vi "Create Client from Template.vi"(7 "Template Library":path, 8 "error in (no error)":errorcluster, 9 "Generated Server Name":string="Generated Server", 10 "Target Project Path":path, 11 "Application ref in":refnum<vi>) -> (0 "error out":errorcluster, 3 "Client library out":refnum<vi>)   [LabVIEW 2019, in "gRPC Template Creation Utility.lvlib"]
uses:
  gRPC Template Creation Utility.lvlib
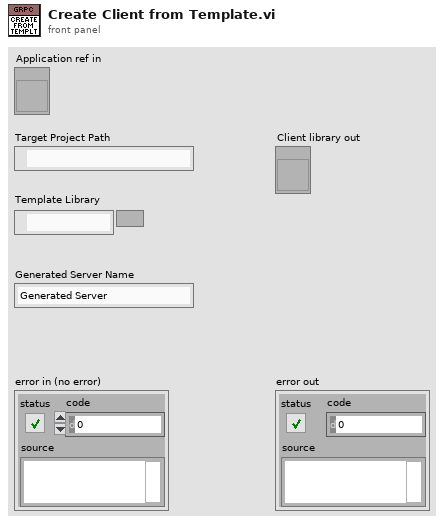
[diagram p1: front panel]
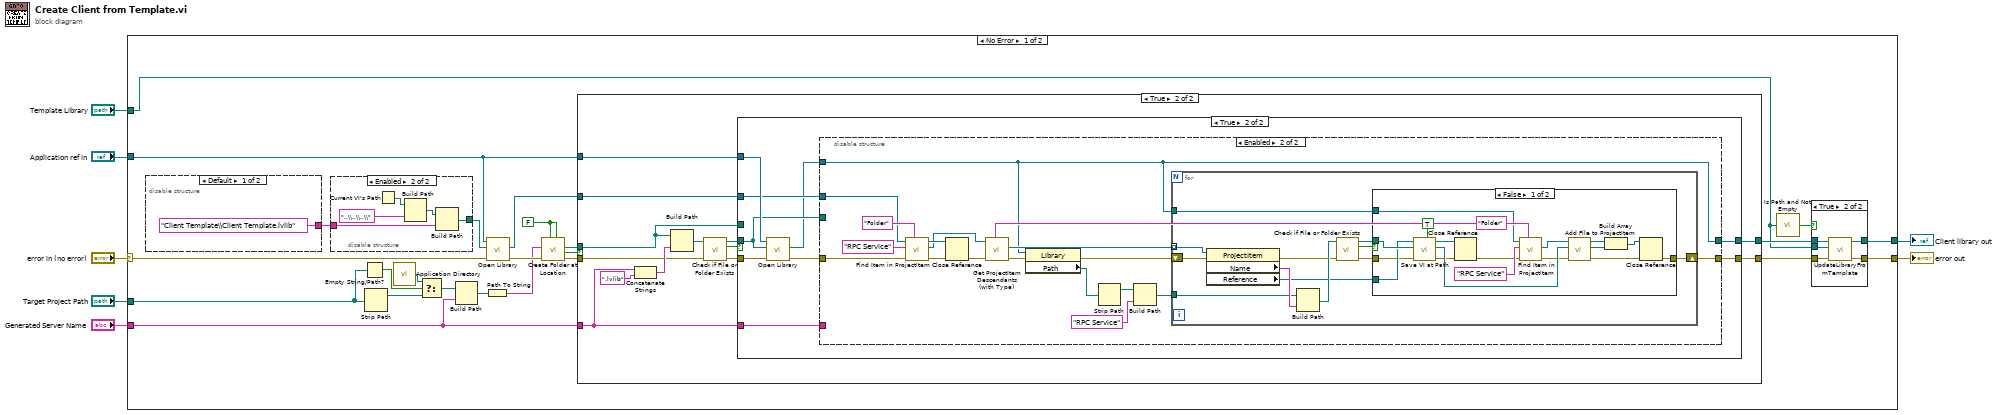
[diagram p0: block diagram]
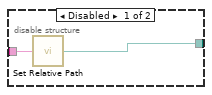
[diagram p3: hidden frame]
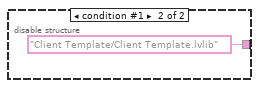
[diagram p4: hidden frame]
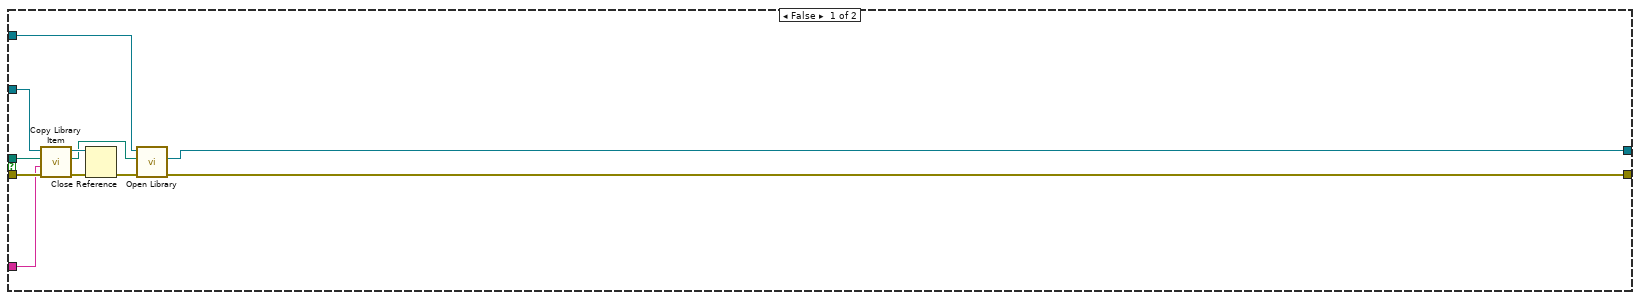
[diagram p5: hidden frame]
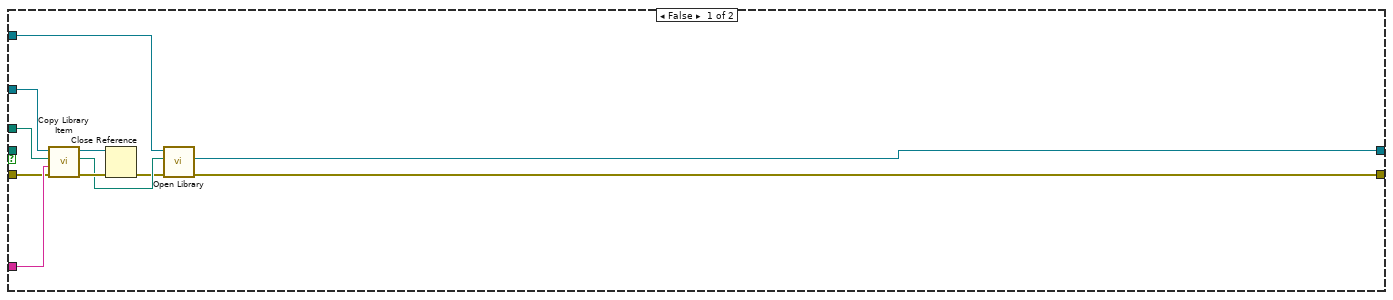
[diagram p6: hidden frame]
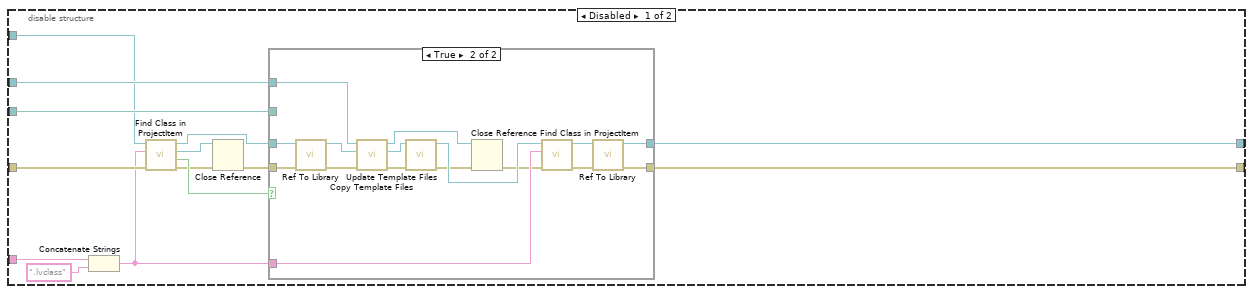
[diagram p7: hidden frame]
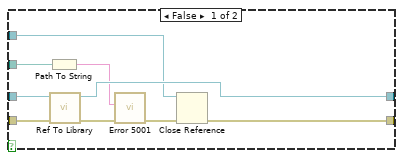
[diagram p8: hidden frame]
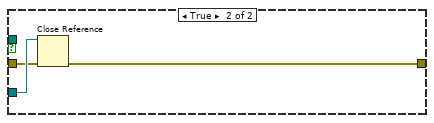
[diagram p9: hidden frame]
diagram:
  n1 = case shown="No Error" "error in (no error)" {
    selector: "error in (no error)" -> [w17 w182]
    tunnel: [w10 w182] -> w7
    tunnel: [w13 _] -> w6
    tunnel: "Target Project Path" -> [w19 _]
    tunnel: "Generated Server Name" -> [w12 _]
    tunnel: "Application ref in" -> [w18 _]
    tunnel: "Template Library" -> [w9 _]
    frame No Error {
      w26 = FALSE ("Use Relative")
      n2 = disable-structure shown="Default" {
        disable-tunnel: ["Client Template\\Client Template.lvlib" ("Application Relative Path") "Client Template/Client Template.lvlib" ("Application Relative Path")] -> w15
        frame condition #0 (active) {
        }
        frame condition #1 {
        }
      }
      n3 = disable-structure shown="Enabled" {
        disable-tunnel: [w40 w43] -> w29
        disable-tunnel: w15 -> [w39 w41]
        frame Disabled {
          n4 = call "Set Relative Path.vi"("Application Relative Path"=w39) -> ("Full Path"=w40:path)
        }
        frame Enabled {
          n5 = Current VI's Path() -> (path=w45:path)
          n6 = Build Path(base path=w45, name or relative path="..\\..\\..\\") -> (appended path=w42:path)
          n7 = Build Path(base path=w42, name or relative path=w41) -> (appended path=w43:path)
        }
      }
      n8 = Empty String/Path?(string/path=w19) -> (empty?=w23:bool)
      n9 = Strip Path(path=w19) -> (stripped path=w22:path)  [unwired: 1 out]
      n10 = call <vilib>:"Application Directory.vi"() -> ("Application Directory"=w20:path)
      n11 = Select(t=w20, s=w23, f=w22) -> (s? t:f=w21:path)
      n12 = Build Path(base path=w21, name or relative path=w12) -> (appended path=w25:path)
      n13 = Path To String(path=w25) -> (string=w24:string)
      n14 = call "Open Library.vi"("error in (no error)"=w17, "Full Path"=w29, "Application in"=w18) -> ("error out"=w30:errorcluster, "Library out"=w27:refnum<vi>)  [unwired: 6 in, 1 out]
      n15 = call "Create Folder at Location.vi"("Override existing (F)"=w26, "Use Relative (F)"=w26, "Error In"=w30, "Path"=w24) -> ("Error Out"=w31:errorcluster, "Already Exists ?"=w16:bool, "Full path out"=w28:path)  [unwired: 5 in]
      n16 = case shown="True" w16 {
        tunnel: [w50 w63] -> w11
        tunnel: [w58 w67] -> w14
        tunnel: w31 -> [w55 w61]
        tunnel: w28 -> [w54 w65]
        tunnel: w27 -> [w53 w66]
        tunnel: w12 -> [w49 w64]
        tunnel: w18 -> [w48 w59]
        frame False {
          n17 = call "Copy Library Item.vi"("error in (no error)"=w55, "Copy Name"=w49, "Copy location"=w54, "Library in"=w53) -> ("error out"=w57:errorcluster, "New Lib Path"=w52:path, "Library out"=w56:refnum<vi>)  [unwired: 5 in]
          n18 = Close Reference(reference=w56, error in (no error)=w57) -> (error out=w51:errorcluster)
          n19 = call "Open Library.vi"("error in (no error)"=w51, "Full Path"=w52, "Application in"=w48) -> ("error out"=w50:errorcluster, "Library out"=w58:refnum<vi>)  [unwired: 6 in, 1 out]
        }
        frame True {
          n20 = Concatenate Strings(w64, ".lvlib" ("string")) -> (w70:string)
          n21 = Build Path(base path=w65, name or relative path=w70) -> (appended path=w69:path)
          n22 = call <vilib>:"Check if File or Folder Exists.vi"("error in (no error)"=w61, "path"=w69) -> ("error out"=w60:errorcluster, "file or folder exists?"=w68:bool, "dup path"=w62:path)  [unwired: 7 in]
          n23 = case shown="True" w68 {
            tunnel: [w73 w89] -> w67
            tunnel: w59 -> [w78 w91]
            tunnel: w66 -> [w77 w86]
            tunnel: w65 -> [w76 _]
            tunnel: w64 -> [w75 w90]
            tunnel: w60 -> [w74 w85]
            tunnel: [w72 w88] -> w63
            tunnel: w62 -> [_ w87]
            frame False {
              n24 = call "Copy Library Item.vi"("error in (no error)"=w74, "Copy Name"=w75, "Copy location"=w76, "Library in"=w77) -> ("error out"=w82:errorcluster, "New Lib Path"=w80:path, "Library out"=w81:refnum<vi>)  [unwired: 5 in]
              n25 = Close Reference(reference=w81, error in (no error)=w82) -> (error out=w79:errorcluster)
              n26 = call "Open Library.vi"("error in (no error)"=w79, "Full Path"=w80, "Application in"=w78) -> ("error out"=w72:errorcluster, "Library out"=w73:refnum<vi>)  [unwired: 6 in, 1 out]
            }
            frame True {
              n27 = call "Open Library.vi"("error in (no error)"=w85, "Full Path"=w87, "Application in"=w91) -> ("error out"=w83:errorcluster, "Library out"=w84:refnum<vi>)  [unwired: 6 in, 1 out]
              n28 = disable-structure shown="Enabled" {
                disable-tunnel: w90 -> [w105 _]
                disable-tunnel: [w104 w135] -> w89
                disable-tunnel: [w103 w133] -> w88
                disable-tunnel: w87 -> [w102 _]
                disable-tunnel: w86 -> [w101 w146]
                disable-tunnel: w84 -> [w100 w135]
                disable-tunnel: w83 -> [w98 w140]
                frame Disabled {
                  n29 = Concatenate Strings(w105, ".lvclass" ("Class Name")) -> (w92:string)
                  n30 = call "Find Class in ProjectItem.vi"("error in (no error)"=w98, "Class Name"=w92, "ProjectItem in"=w100) -> ("error out"=w94:errorcluster, "Found?"=w96:bool, "LVClass out"=w95:refnum<vi>, "ProjectItem out"=w97:refnum<vi>)  [unwired: 5 in]
                  n31 = Close Reference(reference=w95, error in (no error)=w94) -> (error out=w93:errorcluster)
                  n32 = case shown="True" w96 {
                    tunnel: w97 -> [w114 w126]
                    tunnel: [w113 w130] -> w104
                    tunnel: w93 -> [w106 w128]
                    tunnel: [w107 w120] -> w103
                    tunnel: w102 -> [w111 _]
                    tunnel: w101 -> [w110 w119]
                    tunnel: w92 -> [_ w125]
                    frame False {
                      n33 = Path To String(path=w111) -> (string=w109:string)
                      n34 = call "Ref To Library.vi"("error in (no error)"=w106, "ProjectItem in"=w114) -> ("error out"=w112:errorcluster, "Library out"=w113:refnum<vi>)  [unwired: 8 in]
                      n35 = call "Error 5001.vi"("error in (no error)"=w112, "Server Class Path"=w109) -> ("error out"=w108:errorcluster)  [unwired: 9 in]
                      n36 = Close Reference(reference=w110, error in (no error)=w108) -> (error out=w107:errorcluster)
                    }
                    frame True {
                      n37 = call "Ref To Library.vi"("error in (no error)"=w128, "ProjectItem in"=w126) -> ("error out"=w127:errorcluster, "Library out"=w129:refnum<vi>)  [unwired: 8 in]
                      n38 = call "Copy Template Files.vi"("error in (no error)"=w127, "Server Library (Library Item) in"=w129, "Template Library (Library Item) in"=w119) -> ("error out"=w118:errorcluster, "Server Library (Library Item) out"=w117:refnum<vi>, "Template Library (Library Item) out"=w115:refnum<vi>)  [unwired: 6 in]
                      n39 = call "Update Template Files.vi"("error in (no error)"=w118, "Server Library (Library Item) in"=w117) -> ("error out"=w116:errorcluster, "Server Library (Library Item) out"=w124:refnum<vi>)  [unwired: 8 in]
                      n40 = Close Reference(reference=w115, error in (no error)=w116) -> (error out=w122:errorcluster)
                      n41 = call "Find Class in ProjectItem.vi"("error in (no error)"=w122, "Class Name"=w125, "ProjectItem in"=w124) -> ("error out"=w121:errorcluster, "ProjectItem out"=w123:refnum<vi>)  [unwired: 5 in, 2 out]
                      n42 = call "Ref To Library.vi"("error in (no error)"=w121, "ProjectItem in"=w123) -> ("error out"=w120:errorcluster, "Library out"=w130:refnum<vi>)  [unwired: 8 in]
                    }
                  }
                }
                frame Enabled {
                  n43 = call "Find Item in ProjectItem.vi"("Item Type"="Folder", "error in (no error)"=w140, "Name"="RPC Service", "ProjectItem in"=w146) -> ("error out"=w144:errorcluster, "Item Refnum out"=w142:refnum<vi>, "ProjectItem out"=w145:refnum<vi>)  [unwired: 4 in, 1 out]
                  n44 = Close Reference(reference=w145, error in (no error)=w144) -> (error out=w143:errorcluster)
                  n45 = call "Get ProjectItem Descendants (with Type).vi"("Type"="VI", "error in (no error)"=w143, "ProjectItem in"=w142) -> ("error out"=w132:errorcluster, "All Descendents"=w136:refnum<vi>[])  [unwired: 6 in, 1 out]
                  n46 = property class="Library"(reference=w135, error in=w132) -> (error out=w131:errorcluster, "Path"=w139:path)  [unwired: 1 out]
                  n47 = Strip Path(path=w139) -> (stripped path=w138:path)  [unwired: 1 out]
                  n48 = Build Path(base path=w138, name or relative path="RPC Service") -> (appended path=w134:path)
                  n49 = for {
                    tunnel: w136 -> [w160] mode=indexing
                    shift-right: [w150] -> w133
                    shift-left: w131 -> [w149]
                    tunnel: w135 -> [w151]
                    tunnel: w134 -> [w158]
                    n50 = property class="ProjectItem"(reference=w160, error in=w149) -> (error out=w155:errorcluster, "Name"=w159:string, "Reference"=w152:refnum<vi>)  [unwired: 1 out]
                    n51 = Build Path(base path=w158, name or relative path=w159) -> (appended path=w157:path)
                    n52 = call <vilib>:"Check if File or Folder Exists.vi"("error in (no error)"=w155, "path"=w157) -> ("error out"=w154:errorcluster, "file or folder exists?"=w156:bool, "dup path"=w153:path)  [unwired: 7 in]
                    n53 = case shown="False" w156 {
                      tunnel: w154 -> [w165 w180]
                      tunnel: w153 -> [w175 _]
                      tunnel: w152 -> [w174 w181]
                      tunnel: w151 -> [w176 _]
                      tunnel: [w167 w179] -> w150
                      frame False {
                        n54 = call "Save VI at Path.vi"("Save a Copy (F)"=TRUE, "error in (no error)"=w165, "Path"=w175, "VI in"=w174) -> ("error out"=w161:errorcluster, "Path to saved File"=w166:path, "VI out"=w171:refnum<vi>)  [unwired: 5 in]
                        n55 = Close Reference(reference=w171, error in (no error)=w161) -> (error out=w162:errorcluster)
                        n56 = call "Find Item in ProjectItem.vi"("Item Type"="Folder", "error in (no error)"=w162, "Name"="RPC Service", "ProjectItem in"=w176) -> ("error out"=w164:errorcluster, "Item Refnum out"=w172:refnum<vi>)  [unwired: 4 in, 2 out]
                        n57 = call "Add File to ProjectItem.vi"("error in (no error)"=w164, "File Path"=w166, "ProjectItem in"=w172) -> ("error out"=w163:errorcluster, "Added File ref"=w169:refnum<vi>, "ProjectItem out"=w170:refnum<vi>)  [unwired: 6 in]
                        n58 = Build Array(w170, w169) -> (w168:refnum<vi>[])
                        n59 = Close Reference(reference=w168, error in (no error)=w163) -> (error out=w167:errorcluster)
                      }
                      frame True {
                        n60 = Close Reference(reference=w181, error in (no error)=w180) -> (error out=w179:errorcluster)
                      }
                    }
                  }
                }
              }
            }
          }
        }
      }
      n61 = call <vilib>:"Is Path and Not Empty.vi"("path"=w9) -> ("Is Path and Not Empty?"=w8:bool)  [unwired: 4 in]
      n62 = case shown="True" w8 {
        tunnel: w14 -> [w32 w38]
        tunnel: [w32 w37] -> w13
        tunnel: w11 -> [w33 w36]
        tunnel: [w33 w35] -> w10
        tunnel: w9 -> [_ w34]
        frame False {
        }
        frame True {
          n63 = call "UpdateLibraryFromTemplate.vi"("error in (no error)"=w36, "Prototype Library Path"=w34, "Target Library"=w38) -> ("error out"=w35:errorcluster, "Target Library Out"=w37:refnum<vi>)  [unwired: 7 in]
        }
      }
    }
    frame Error {
    }
  }
  "error out" <- w7
  "Client library out" <- w6
